vi "GetSetFrameCount.vi"(7 "Set":bool, 8 "error in (no error)":errorcluster, 10 "Frame Count":i64, 11 "Camera in":refnum<class "Camera.lvclass">) -> (0 "error out":errorcluster, 2 "Frame Count":i64)   [LabVIEW 2020, in "Camera.lvclass"]
uses:
  Camera.lvclass
  Camera.lvclass/Camera.ctl
  bin/gindustrialcam_32-1.dll
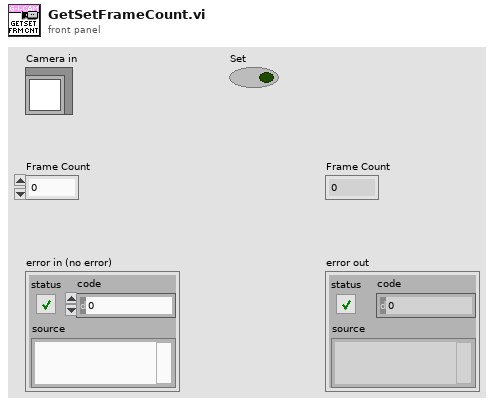
[diagram p1: front panel]
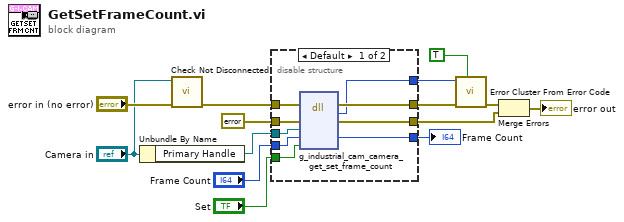
[diagram p0: block diagram]
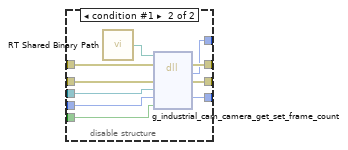
[diagram p2: hidden frame]
diagram:
  n1 = Unbundle By Name("Camera in") -> ("Primary Handle"=w5:refnum<data-value>)
  n2 = call "Check Not Disconnected.vi"("error in (no error)"="error in (no error)", "Camera in"="Camera in") -> ("error out"=w4:errorcluster)  [unwired: 9 in]
  n3 = disable-structure shown="Default" {
    disable-tunnel: [w23 w33] -> w14
    disable-tunnel: "Set" -> [w22 w32]
    disable-tunnel: "Frame Count" -> [w21 w31]
    disable-tunnel: [w20 w30] -> w11
    disable-tunnel: [w19 w29] -> w10
    disable-tunnel: [w18 w28] -> w8
    disable-tunnel: errorcluster {"status"=FALSE, "code"=0, "source"=""} ("error constant") -> [w17 w27]
    disable-tunnel: w5 -> [w16 w26]
    disable-tunnel: w4 -> [w15 w25]
    frame condition #0 (active) {
      n4 = dll-call lib="C:/serenial/lib/g-industrial-camera/LabVIEW/g_industrial_cam/bin/gindustrialcam_*-1.*" fn="g_industrial_cam_camera_get_set_frame_count"(error in=w15, "err"=w17, "edvr"=w16, "count"=w21, "set"=w22) -> (error out=w20:errorcluster, "Mg_Error"=w19:i32, "err"=w18:errorcluster, "count"=w23:i64)  [unwired: 4 in, 1 out]
    }
    frame condition #1 {
      n5 = call "RT Shared Binary Path.vi"() -> ("Path"=w24:path)
      n6 = dll-call lib="C:/serenial/lib/g-industrial-camera/LabVIEW/g_industrial_cam/bin/gindustrialcam_*-1.*" fn="g_industrial_cam_camera_get_set_frame_count"(path in=w24, error in=w25, "err"=w27, "edvr"=w26, "count"=w31, "set"=w32) -> (error out=w30:errorcluster, "Mg_Error"=w29:i32, "err"=w28:errorcluster, "count"=w33:i64)  [unwired: 3 in, 1 out]
    }
  }
  "Frame Count" <- w14
  n7 = call <vilib>:"Error Cluster From Error Code.vi"("show call chain? (False)"=TRUE, "error in (no error)"=w11, "error code (0)"=w10) -> ("error out"=w9:errorcluster)  [unwired: 6 in]
  n8 = Merge Errors(w9, w8) -> (→"error out":errorcluster)
